vi "Arm Control (FPGA).vi"() -> ()   [LabVIEW 2016]
uses:
  <vilib>/rvi/Emulation/niFpgaSctlEmulationGetInTimedLoop.vi
  <vilib>/rvi/Emulation/niFpgaProcessEmulError.vi
  <vilib>/rvi/eio/common/nirviEmuTemplateMethod_errors.vi
  <vilib>/rvi/Emulation/niFpgaGetClockAttributes.vi
  <vilib>/rvi/Emulation/niFpgaEmulationReportErrorSimple.vi
  <vilib>/robotics/Utilities/FPGA Utilities/Generate Digital Pulse (uSec).vi
  <vilib>/rvi/Emulation/niFpgaCriticalErrorInLSC.vi
  <vilib>/eio/EIONode/EIONode.xnode
  <vilib>/robotics/Utilities/FPGA Utilities/NI_Robotics_FPGA Utilities.lvlib
panel:
  out "ConnectorC/DIO3":bool
  out "ConnectorC/DIO1":bool
  in  "Motor Direction":bool
  in  "Motor Power":u32(slide) scale=0.0..1000.0
  in  "S 6":bool
  in  "S 5":bool
  in  "S 4":bool
  in  "Servo 6":u32(slide) scale=0.0..3000.0
  in  "Servo 5":u32(slide) scale=0.0..3000.0
  in  "stop":bool
  in  "Servo 4":u32(slide) scale=0.0..3000.0
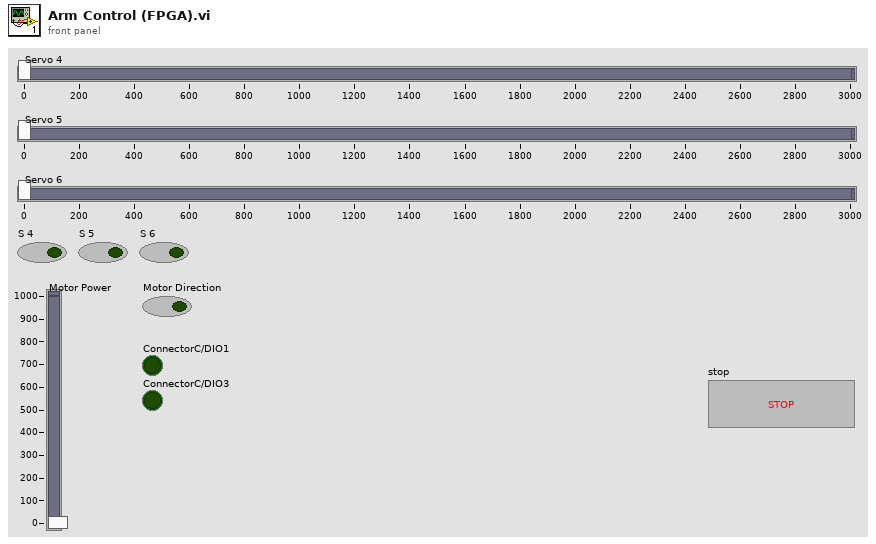
[diagram p1: front panel]
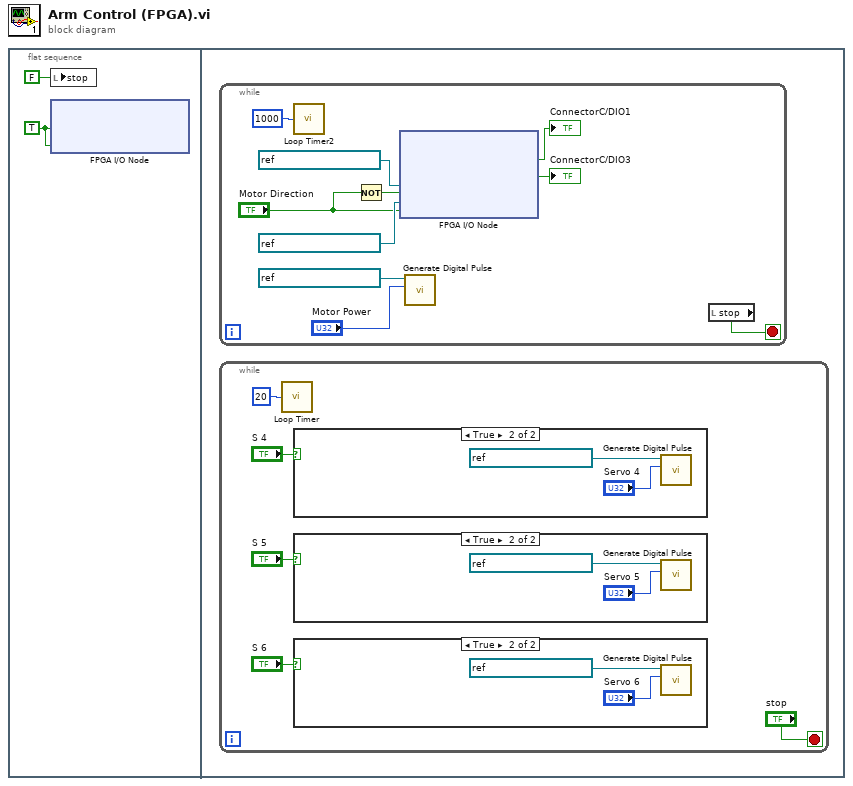
[diagram p0: block diagram]
diagram:
  n1 = flat-sequence {
    frame #0 {
      w1 = TRUE ("ConnectorC/DIO0")
      n2 = local write "stop"(FALSE ("stop")) -> ()
      n3 = xnode "FPGA I/O Node"("ConnectorC/DIO0"=w1, "ConnectorC/DIO2"=w1) -> ()  [unwired: 2 in, 2 out]
    }
    frame #1 {
      n4 = while {
        stop <- w5 stop-if-true
        n5 = call "Loop Timer2"("Count(uSec)"=u32 1000) -> ()  [unwired: 1 out]
        n6 = Not(x="Motor Direction") -> (.not. x?=w4:bool)
        n7 = xnode "FPGA I/O Node"("I/O Item"=w4, "FPGA I/O In"=refnum<k21> "ConnectorB/DIO2", "I/O Item"="Motor Direction", "FPGA I/O In"=refnum<k21> "ConnectorB/DIO3") -> ("ConnectorC/DIO1"=→"ConnectorC/DIO1":bool, "ConnectorC/DIO3"=→"ConnectorC/DIO3":bool)  [unwired: 2 in, 4 out]
        n8 = call-poly <vilib>:"Generate Digital Pulse.vi"("pulse width (uSec)"="Motor Power", "FPGA digital output"=refnum<k21> "ConnectorB/DIO4") -> ()  [unwired: 10 in]
        n9 = local read "stop"() -> (w5:bool)
      }
      n10 = while {
        stop <- "stop" stop-if-true
        n11 = call "Loop Timer"("Count(mSec)"=u32 20) -> ()  [unwired: 1 out]
        n12 = case shown="True" "S 4" {
          frame False {
          }
          frame True {
            n13 = call-poly <vilib>:"Generate Digital Pulse.vi"("pulse width (uSec)"="Servo 4", "FPGA digital output"=refnum<k21> "ConnectorC/DIO4") -> ()  [unwired: 10 in]
          }
        }
        n14 = case shown="True" "S 5" {
          frame False {
          }
          frame True {
            n15 = call-poly <vilib>:"Generate Digital Pulse.vi"("pulse width (uSec)"="Servo 5", "FPGA digital output"=refnum<k21> "ConnectorC/DIO5") -> ()  [unwired: 10 in]
          }
        }
        n16 = case shown="True" "S 6" {
          frame False {
          }
          frame True {
            n17 = call-poly <vilib>:"Generate Digital Pulse.vi"("pulse width (uSec)"="Servo 6", "FPGA digital output"=refnum<k21> "ConnectorC/DIO6") -> ()  [unwired: 10 in]
          }
        }
      }
    }
  }
